vi "YAV_Close.vi"(10 "error in":errorcluster, 11 "Device ID":u16) -> (3 "error out":errorcluster caption="错误输出")   [LabVIEW 2020]
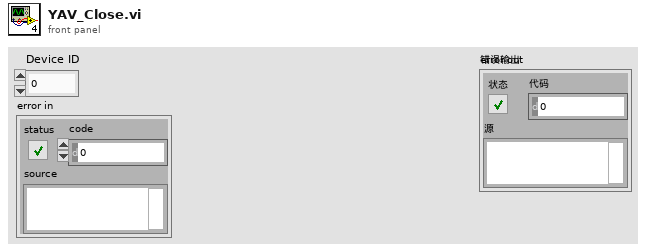
[diagram p1: front panel]
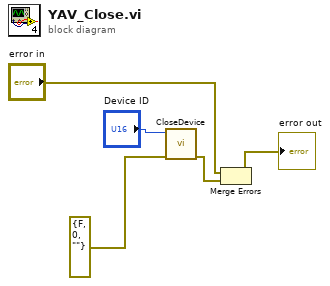
[diagram p0: block diagram]
diagram:
  n1 = call "CloseDevice.vi"("error in (no error)"=errorcluster {"status"=FALSE, "code"=0, "source"=""}, "id"="Device ID") -> ("错误输出"=w4:errorcluster)  [unwired: 9 in]
  n2 = Merge Errors("error in", w4) -> (→"error out":errorcluster)
